vi "LTE set UL Channel.vi"(8 "error in (no error)":errorcluster caption="에러 입력(에러 없음)", 10 "UL Channel":i32, 11 "Instrument Manager 입력":refnum<class "Instrument Manager.lvclass">) -> (0 "error out":errorcluster caption="에러 출력", 3 "Instrument Manager 출력":refnum<class "Instrument Manager.lvclass">)   [LabVIEW 2023, in "Instrument Manager.lvclass"]
uses:
  Instrument Manager.lvclass
  Module/ANRITSU Call Box/Type Definition/LTE Uplink Channel Number Info.ctl
  Module/ANRITSU Call Box/Type Definition/LTE Uplink Channel Number Target.ctl
  Instrument Manager.lvclass/Instrument Manager.ctl
  Module/ANRITSU Call Box/Interface Class/Anritsu Call Box.lvclass
  Module/ANRITSU Call Box/ANRITSU Call Box.lvlib
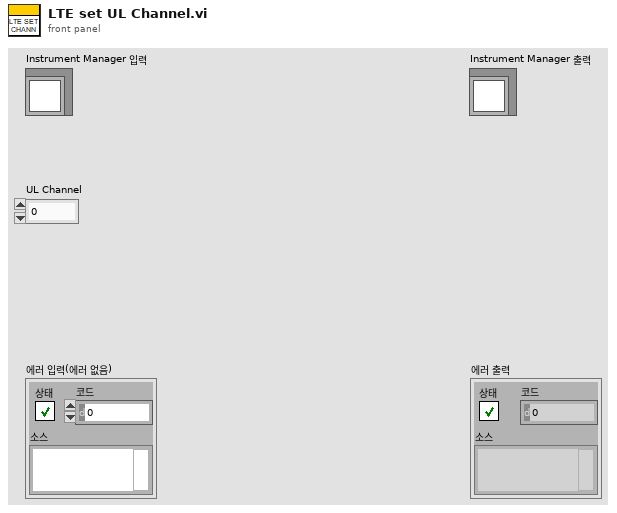
[diagram p1: front panel]
types:
  T1 = typedef "ANRITSU Call Box.lvlib/LTE Uplink Channel Number Target.ctl" = enum16{"PCC Uplink", "SCC-1 Uplink", "All"}
  T2 = typedef "ANRITSU Call Box.lvlib/LTE Uplink Channel Number Info.ctl" = cluster{"PCC Uplink":i32, "SCC-1 Uplink":i32}
  T3 = cluster{"Anritsu Call Box":refnum<class "Anritsu Call Box.lvclass">, "Spectrum Analyzer":refnum<class "Interface_Spectrum.lvclass">, "RF Switch Box":refnum<class "RF Filter Box.lvclass">, "Turn Table":refnum<class "Interface - Turn Table.lvclass">, "Mast":refnum<class "Interface - Mast.lvclass">, "3D Controller":refnum<class "Interface_3D Controller.lvclass">}
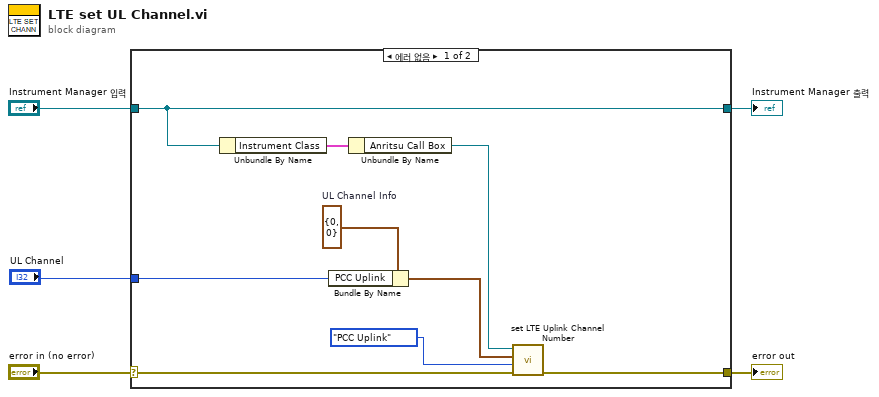
[diagram p0: block diagram]
diagram:
  n1 = case shown="에러 없음" "error in (no error)" {
    selector: "error in (no error)" -> [w9 w16]
    tunnel: [w8 w16] -> w4
    tunnel: [w14 w15] -> w2
    tunnel: "Instrument Manager 입력" -> [w14 w15]
    tunnel: "UL Channel" -> [w6 _]
    frame No Error {
      w11 = T2 {"PCC Uplink"=0, "SCC-1 Uplink"=0}  # UL Channel Info
      n2 = Unbundle By Name(w14) -> ("Instrument Class"=w13:T3)
      n3 = Bundle By Name(cluster=w11, "PCC Uplink"=w6) -> (w7:T2)
      n4 = Unbundle By Name(w13) -> ("Anritsu Call Box"=w12:refnum<class "Anritsu Call Box.lvclass">)
      n5 = call-dynamic "set LTE Uplink Channel Number.vi"("error in (no error)"=w9, "UL Channel Arguments"=LTE_Uplink_Channel_Number_Target."PCC Uplink", "UL Channel Info"=w7, "Anritsu Call Box in"=w12) -> ("error out"=w8:errorcluster)  [unwired: 6 in, 1 out]
    }
    frame Error {
    }
  }
  "error out" <- w4
  "Instrument Manager 출력" <- w2
